vi "Drive Controller.vi"(8 "error in":errorcluster) -> ()   [LabVIEW 2025]
doc: "This VI executes continuously carrying out the current operation and responding to updates or new operation requests. It will often contain the timing or control code that is difficult to place directly in TeleOp. This VI generally opens all sensors and motors and isolates the rest of the robot code from knowing implementation details of how the operations are carried out."
uses:
  <vilib>/Rock Robotics/WPI/Framework/Completion Status.ctl
  Drive Setpoints.ctl
  Drive Operations.ctl
  bordeaux-main/Bordeaux/Types/Single Cmd Info.ctl
  <vilib>/picture/picture.llb/imagedata.ctl
  bordeaux-main/Bordeaux/Types/Trajectory Data.ctl
  bordeaux-main/Bordeaux/Types/Segment Type.ctl
  <vilib>/Rock Robotics/WPI/ThirdParty/REV Robotics/REVLib/Typedef/SPARK PID Gains.ctl
  <vilib>/Rock Robotics/WPI/ThirdParty/REV Robotics/REVLib/Typedef/SPARK Feed Forward Gains.ctl
  <vilib>/Rock Robotics/WPI/ThirdParty/REV Robotics/REVLib/Typedef/Spark MAX Idle Mode.ctl
  <vilib>/Rock Robotics/WPI/ThirdParty/REV Robotics/REVLib/Typedef/Spark MAX Control Type.ctl
  <vilib>/Rock Robotics/WPI/ThirdParty/REV Robotics/REVLib/SubVI/Public/SPARK Open Brushless.vi
  <vilib>/Rock Robotics/WPI/ThirdParty/REV Robotics/REVLib/SubVI/Public/SPARK Configure Power Current Limit.vi
  <vilib>/Rock Robotics/WPI/ThirdParty/REV Robotics/REVLib/SubVI/Public/SPARK Configure Follower Mode From Ref.vi
  <vilib>/Rock Robotics/WPI/ThirdParty/REV Robotics/REVLib/SubVI/Public/SPARK Configure Basic Idle Mode.vi
  <vilib>/Rock Robotics/WPI/ThirdParty/REV Robotics/REVLib/SubVI/Public/SPARK Configure Closed Loop Gains.vi
panel:
  in  "Feed Forward Gains":T1={"kV"=0.00205, "kS"=0.0, "kA"=0.01, "kG"=0.0, "kCos"=0.0, "kCosRatio"=0.0}
  in  "PID Gains":T2={"kP"=1e-05, "kI"=0.0, "kD"=0.0}
  in  "V Scale":dbl=1.0
  in  "Interactive Values":T3
  in  "Buttons":cluster{"Execute Cmd":bool, "Abort Cmd":bool}
  out "Command Timing":cluster{"Start Time (ms)":u32, "Iterations":i32}
  out "Status":T9
  out "Setpoints":T10(graph)
  out "Current\nCmd":string
  # "Interactive Command: You may fill in the settings for a command\nand schedule it with the Execute button. You can observe and abort\nany command while fine tuning the code for the controller."
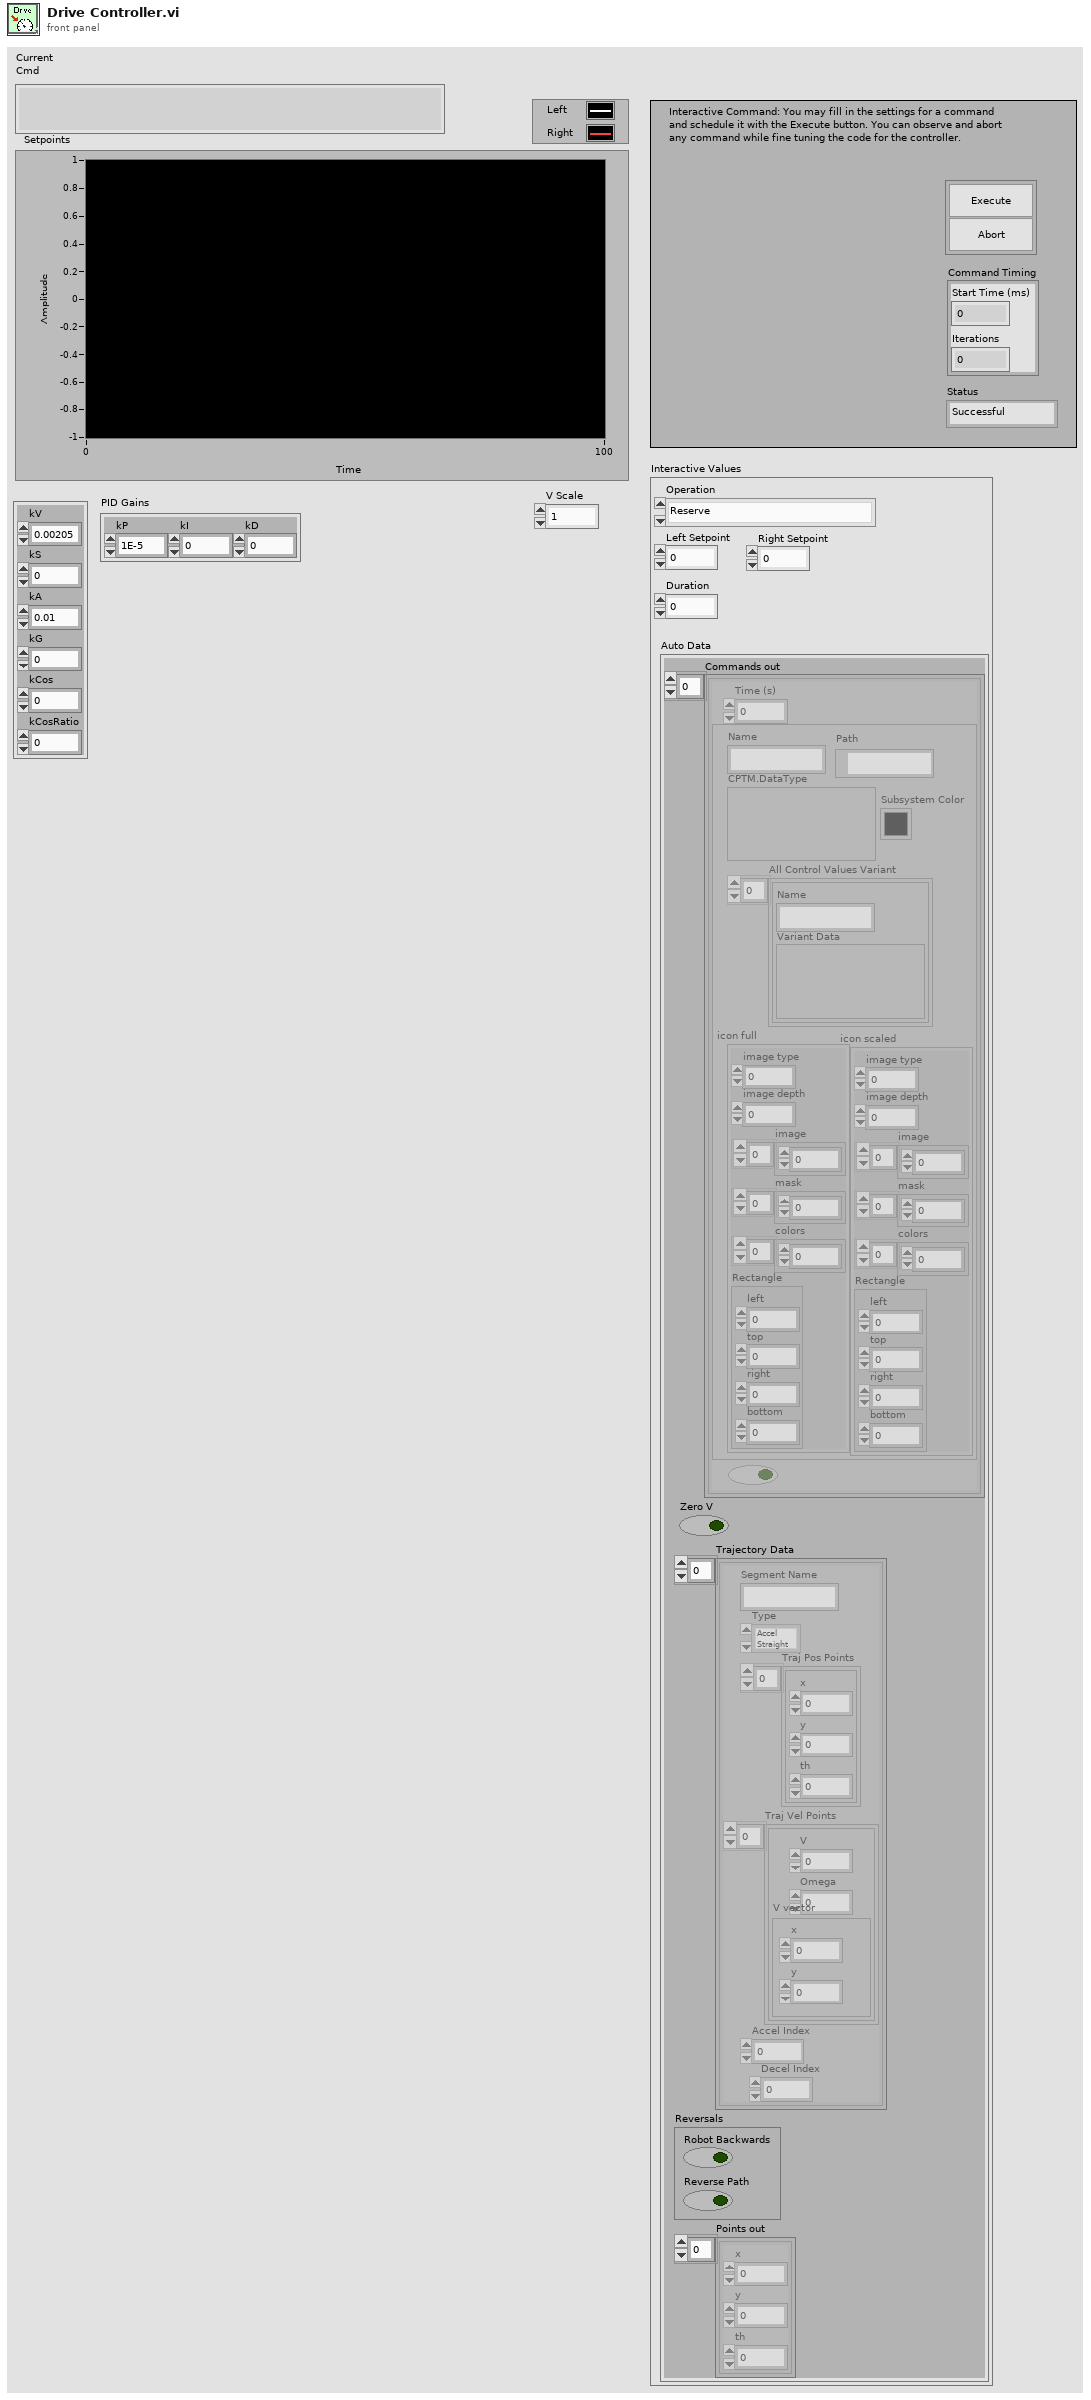
[diagram p1: front panel]
types:
  T1 = typedef "SPARK Feed Forward Gains.ctl" = cluster{"kV":dbl, "kS":dbl, "kA":dbl, "kG":dbl, "kCos":dbl, "kCosRatio":dbl}
  T2 = typedef "SPARK PID Gains.ctl" = cluster{"kP":dbl, "kI":dbl, "kD":dbl}
  T3 = typedef "Drive Setpoints.ctl" = cluster{"Operation":T4, "Left Setpoint":dbl, "Right Setpoint":dbl, "Duration":dbl, "Auto Data":cluster{"Commands out":cluster{"Time (s)":dbl, T5, bool}[], "Zero V":bool, "Trajectory Data":T7, "Reversals":cluster{"Robot Backwards":bool, "Reverse Path":bool}, "Points out":cluster{"x":dbl, "y":dbl, "th":dbl}[]}}
  T4 = typedef "Drive Operations.ctl" = enum16{"Reserve", "Read Current", "Immediate", "Drive for Time", "Play Path", "Drive for Distance", "Turn Aligning"}
  T5 = typedef "Single Cmd Info.ctl" = cluster{"Name":string, "CPTM.DataType":variant, "All Control Values Variant":cluster{"Name":string, "Variant Data":variant}[], "icon full":T6, "icon scaled":T6, "Path":path, "Subsystem Color":u32}
  T6 = typedef "imagedata.ctl" = cluster{"image type":i32, "image depth":i32, "image":u8[], "mask":u8[], "colors":u32[], "Rectangle":cluster{"left":i16, "top":i16, "right":i16, "bottom":i16}}
  T7 = typedef "Trajectory Data.ctl" = cluster{"Segment Name":string, "Type":T8, "Traj Pos Points":cluster{"x":dbl, "y":dbl, "th":dbl}[], "Traj Vel Points":cluster{"V":dbl, "Omega":dbl, "V vector":cluster{"y":dbl, "x":dbl}}[], "Accel Index":i32, "Decel Index":i32}[]
  T8 = typedef "Segment Type.ctl" = enum16{"Accel Straight", "Const Straight", "Blend", "Circle", "Bezier"}
  T9 = typedef "Completion Status.ctl" = enum16{"Successful", "Aborted", "Incomplete"}
  T10 = cluster{"Left Setpoint":dbl, "Right Setpoint":dbl}
  T11 = typedef "Spark MAX Idle Mode.ctl" = enum16{"Coast", "Brake"}
  T12 = typedef "WPI_MotorControlDeviceRef.ctl" = cluster{"DeviceStatus":errorcluster, "Type":T13, "PWM":cluster{"PWM Channel":T14, "DeadBand":T15}, "CAN":cluster{"Device Number":u8, "SetOutput VI Ref":variant, "GetOutput VI Ref":variant, "Enable VI Ref":variant, "Disable VI Ref":variant, "Data":variant}, "Invert":bool, "DIO PWM":cluster{"PWM \"Enable\" Channel":T14, "DIOChannel":T16, "PWM Rate":dbl}}
  T13 = typedef "WPI_MotorControlType.ctl" = enum16{"PWM", "CAN", "DIO PWM"}
  T14 = typedef "FPGA_DIOPWMChannel.ctl" = enum8{"PWM 0", "PWM 1", "PWM 2", "PWM 3", "PWM 4", "PWM 5", "PWM 6", "PWM 7", "PWM 8", "PWM 9", "PWM MXP 0", "PWM MXP 1", "PWM MXP 2", "PWM MXP 3", "PWM MXP 4", "PWM MXP 5", "PWM MXP 6", "PWM MXP 7", "PWM MXP 8", "PWM MXP 9", "Invalid"}
  T15 = typedef "WPI_PWMDeadband.ctl" = cluster{"Name":string, "maxPositivePwm":i32, "minPositivePwm":i32, "centerPwm":i32, "maxNegativePwm":i32, "minNegativePwm":i32, "angularRange":u16}
  T16 = typedef "FPGA_DIOChannel.ctl" = enum8{"DIO 0", "DIO 1", "DIO 2", "DIO 3", "DIO 4", "DIO 5", "DIO 6", "DIO 7", "DIO 8", "DIO 9", "DIO MXP 0", "DIO MXP 1", "DIO MXP 2", "DIO MXP 3", "DIO MXP 4", "DIO MXP 5", "DIO MXP 6", "DIO MXP 7", "DIO MXP 8", "DIO MXP 9", "DIO MXP 10", "DIO MXP 11", "DIO MXP 12", "DIO MXP 13", "DIO MXP 14", "DIO MXP 15", "SPI Port CS1", "SPI Port CS2", "SPI Port CS3", "SPI Port MISO", "SPI Port MOSI", "Invalid"}
  T17 = typedef "Command Status Info.ctl" = cluster{"Name":string, "Status":T9, "notifier out":T18}
  T18 = typedef "Completion Notifier.ctl" = refnum<notifier>
  T19 = cluster{"SubSystem Data":T3, cluster{"Start Time (ms)":u32, "Iterations":i32}, cluster{"Command Info":T17, "Description":string, "Default Command":T3, "queue out":refnum<queue>, "Subsystem Name":string}}
  T20 = cluster{"Commands out":cluster{"Time (s)":dbl, T5, bool}[], "Zero V":bool, "Trajectory Data":T7, "Reversals":cluster{"Robot Backwards":bool, "Reverse Path":bool}, "Points out":cluster{"x":dbl, "y":dbl, "th":dbl}[]}
  T21 = typedef "Spark MAX Control Type.ctl" = enum16{"Percent VBus", "Voltage", "Velocity", "Position", "Smart Motion", "Current", "Smart Velocity", "MAXMotion Position", "MAXMotion Velocity"}
  T22 = cluster{"SubSystem Data":T3, cluster{"Start Time (ms)":u32, "Iterations":i32}, "Default Command Arguments":cluster{"Command Info":T17, "Description":string, "Default Command":T3, "queue out":refnum<queue>, "Subsystem Name":string}}
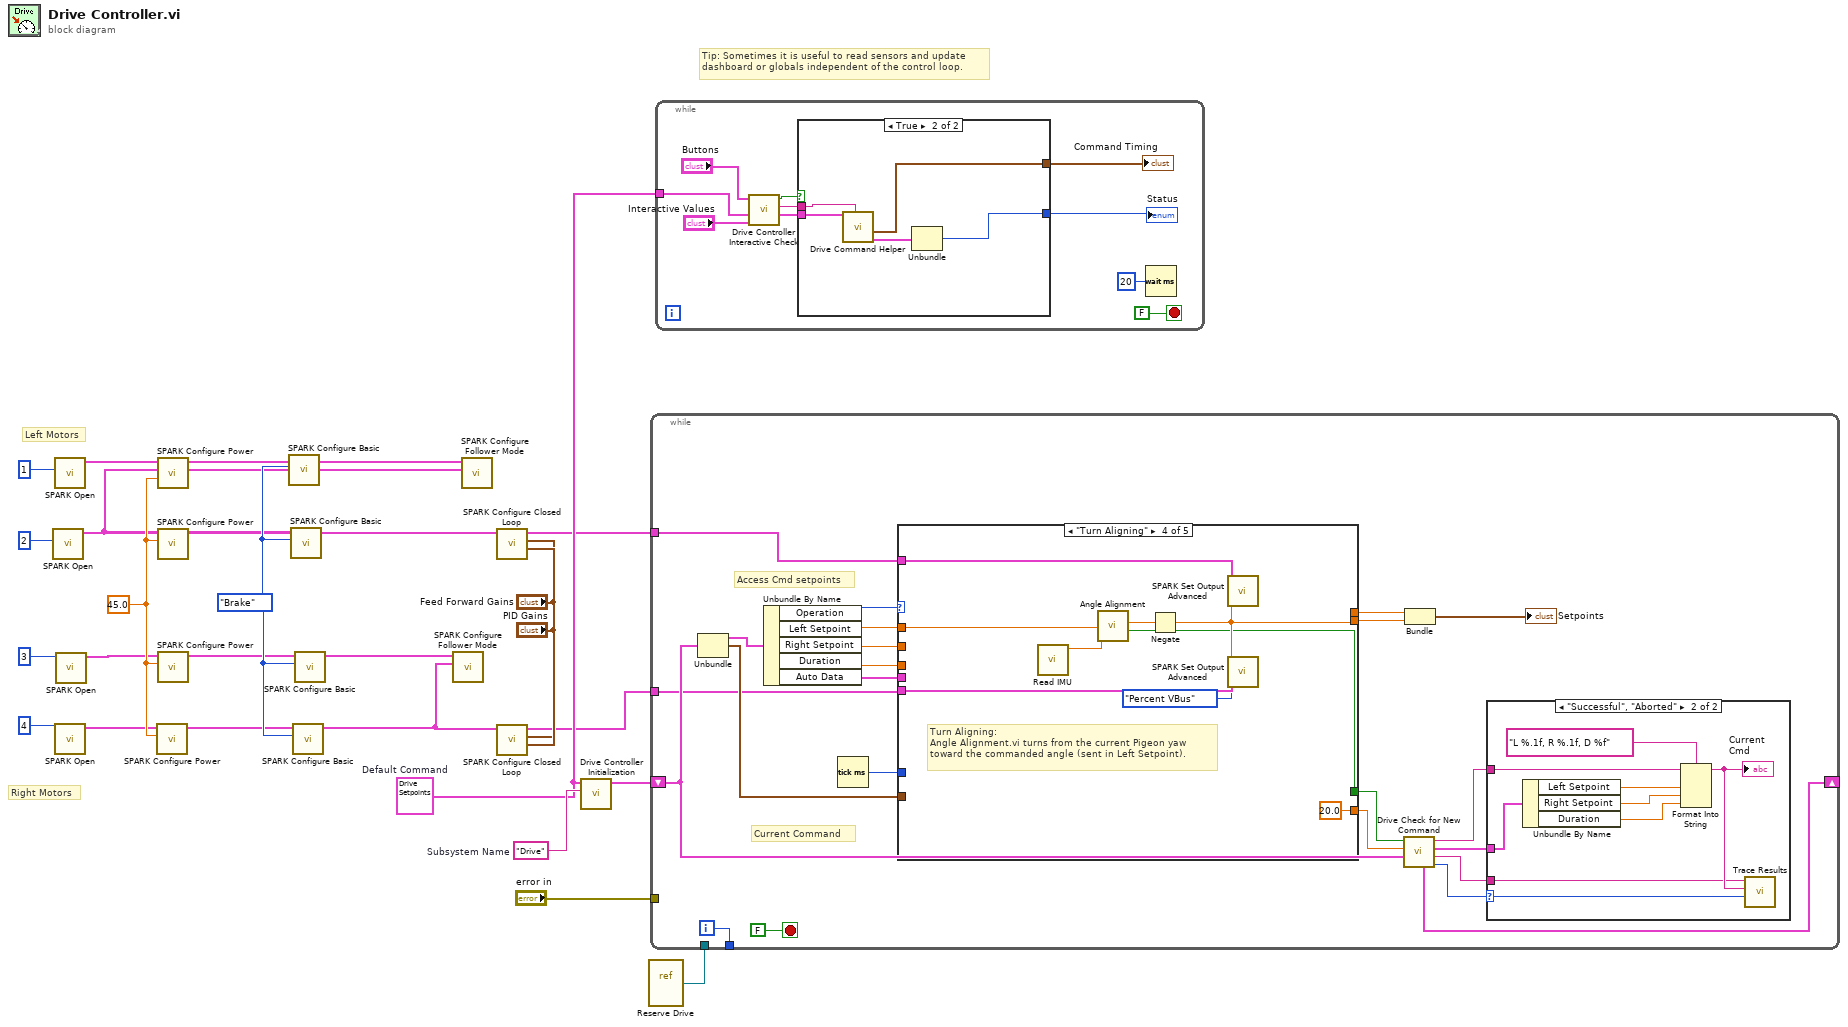
[diagram p0: block diagram]
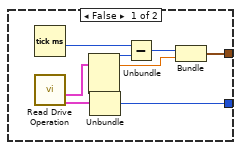
[diagram p2: hidden frame]
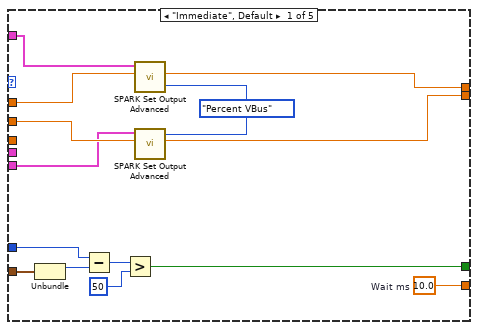
[diagram p4: hidden frame]
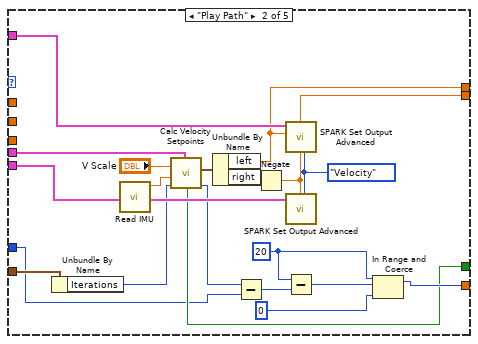
[diagram p5: hidden frame]
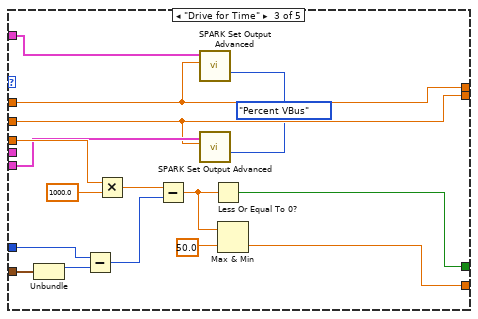
[diagram p6: hidden frame]
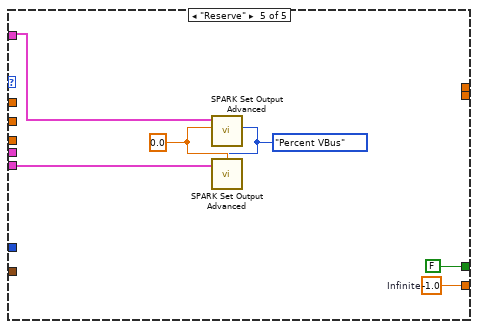
[diagram p7: hidden frame]
diagram:
  w7 = Spark_MAX_Idle_Mode."Brake" ("Idle Mode")
  w8 = 45.0 ("Primay Current Limit (80A)")
  w13 = T3 {"Operation"=enum."Reserve", "Left Setpoint"=0.0, "Right Setpoint"=0.0, "Duration"=0.0, "Auto Data"={"Commands out"=[], "Zero V"=FALSE, "Trajectory Data"=[], "Reversals"={"Robot Backwards"=FALSE, "Reverse Path"=FALSE}, "Points out"=[]}}  # Default Command
  w17 = "Drive"  # Subsystem Name
  # "Right Motors"
  # "Left Motors"
  # "Tip: Sometimes it is useful to read sensors and update\ndashboard or globals independent of the control loop."
  n1 = call-poly <vilib>:"SPARK Open.vi"("Device Number"=u8 2) -> ("MotorControlDeviceRef"=w2:T12)  [unwired: 9 in, 1 out]
  n2 = call-poly <vilib>:"SPARK Open.vi"("Device Number"=u8 1) -> ("MotorControlDeviceRef"=w1:T12)  [unwired: 9 in, 1 out]
  n3 = call-poly <vilib>:"SPARK Open.vi"("Device Number"=u8 4) -> ("MotorControlDeviceRef"=w3:T12)  [unwired: 9 in, 1 out]
  n4 = call-poly <vilib>:"SPARK Open.vi"("Device Number"=u8 3) -> ("MotorControlDeviceRef"=w4:T12)  [unwired: 9 in, 1 out]
  n5 = call-poly <vilib>:"SPARK Configure Power.vi"("Current Limit A (100)"=w8, "MotorControlDeviceRef in"=w3) -> ()  [unwired: 8 in, 2 out]
  n6 = call-poly <vilib>:"SPARK Configure Power.vi"("Current Limit A (100)"=w8, "MotorControlDeviceRef in"=w1) -> ()  [unwired: 8 in, 2 out]
  n7 = call-poly <vilib>:"SPARK Configure Power.vi"("Current Limit A (100)"=w8, "MotorControlDeviceRef in"=w2) -> ()  [unwired: 8 in, 2 out]
  n8 = call-poly <vilib>:"SPARK Configure Power.vi"("Current Limit A (100)"=w8, "MotorControlDeviceRef in"=w4) -> ()  [unwired: 8 in, 2 out]
  n9 = call-poly <vilib>:"SPARK Configure Basic.vi"("Idle Mode"=w7, "MotorControlDeviceRef in"=w1) -> ()  [unwired: 8 in, 2 out]
  n10 = call-poly <vilib>:"SPARK Configure Basic.vi"("Idle Mode"=w7, "MotorControlDeviceRef in"=w2) -> ()  [unwired: 8 in, 2 out]
  n11 = call-poly <vilib>:"SPARK Configure Basic.vi"("Idle Mode"=w7, "MotorControlDeviceRef in"=w3) -> ()  [unwired: 8 in, 2 out]
  n12 = call-poly <vilib>:"SPARK Configure Basic.vi"("Idle Mode"=w7, "MotorControlDeviceRef in"=w4) -> ()  [unwired: 8 in, 2 out]
  n13 = call-poly <vilib>:"SPARK Configure Follower Mode.vi"("Leader MotorControlDeviceRef"=w3, "MotorControlDeviceRef in"=w4) -> ()  [unwired: 8 in, 2 out]
  n14 = call-poly <vilib>:"SPARK Configure Follower Mode.vi"("Leader MotorControlDeviceRef"=w2, "MotorControlDeviceRef in"=w1) -> ()  [unwired: 8 in, 2 out]
  n15 = call-poly <vilib>:"SPARK Configure Closed Loop.vi"("Feed Forward Gains"="Feed Forward Gains", "PID Gains"="PID Gains", "MotorControlDeviceRef in"=w2) -> ()  [unwired: 7 in, 2 out]
  n16 = call-poly <vilib>:"SPARK Configure Closed Loop.vi"("Feed Forward Gains"="Feed Forward Gains", "PID Gains"="PID Gains", "MotorControlDeviceRef in"=w3) -> ()  [unwired: 7 in, 2 out]
  n17 = call "Drive Controller Initialization.vi"("Subsystem Name"=w17, "Default Command"=w13) -> ("Current Command"=w15:T19)  [unwired: 9 in]
  n18 = vi-ref "Reserve Drive.vi"() -> (w14:refnum<vi>)
  n19 = while {
    shift-right: [w28] -> _
    shift-left: w15 -> [w21]
    tunnel: [w39] -> _
    tunnel: "error in" -> [_]
    tunnel: w14 -> [_]
    tunnel: w2 -> [w20]
    tunnel: w3 -> [w19]
    i -> [w39]
    stop <- FALSE stop-if-true
    # "Current Command"
    # "Access Cmd setpoints"
    n20 = Unbundle(w21) -> ("SubSystem Data"=w35:T3, w22:cluster{"Start Time (ms)":u32, "Iterations":i32})  [unwired: 1 out]
    n21 = Unbundle By Name(w35) -> ("Operation"=w34:T4, "Left Setpoint"=w33:dbl, "Right Setpoint"=w32:dbl, "Duration"=w31:dbl, "Auto Data"=w18:T20)
    n22 = Tick Count (ms)() -> (millisecond timer value=w30:u32)
    n23 = case shown="\"Turn Aligning\"" w34 {
      tunnel: [w61 w76 w87 20.0 ("Infinite") w112] -> w27
      tunnel: [w56 w68 w92 w100 FALSE ("ignore previous (F)")] -> w26
      tunnel: w22 -> [w55 w81 w94 _ _]
      tunnel: [w53 w72 w85 w103 _] -> w37
      tunnel: [w52 w70 w83 w103 _] -> w36
      tunnel: w33 -> [w53 _ w85 w105 _]
      tunnel: w32 -> [w52 _ w83 _ _]
      tunnel: w31 -> [_ _ w91 _ _]
      tunnel: w30 -> [w57 w62 w90 _ _]
      tunnel: w20 -> [w54 w75 w86 w102 w110]
      tunnel: w19 -> [w51 w74 w84 w101 w109]
      tunnel: w18 -> [_ w69 _ _ _]
      frame "Immediate", Default {
        w50 = Spark_MAX_Control_Type."Percent VBus" ("Control Mode")
        w61 = 10.0  # Wait ms
        n24 = Unbundle(w55) -> ("Start Time (ms)"=w58:u32)  [unwired: 1 out]
        n25 = Subtract(x=w57, y=w58) -> (x-y=w59:u32)
        n26 = Greater?(x=w59, y=u8 50 ("Left Motor")) -> (0:w56:bool)
        n27 = call <vilib>:"SPARK Set Output Advanced.vi"("Control Mode"=w50, "Setpoint"=w53, "MotorControlDevRef"=w54) -> ()  [unwired: 7 in, 2 out]
        n28 = call <vilib>:"SPARK Set Output Advanced.vi"("Control Mode"=w50, "Setpoint"=w52, "MotorControlDevRef"=w51) -> ()  [unwired: 7 in, 2 out]
      }
      frame "Play Path" {
        w73 = Spark_MAX_Control_Type."Velocity" ("Control Mode")
        w78 = u32 20 ("x")
        n29 = Unbundle By Name(w81) -> ("Iterations"=w66:i32)
        n30 = call "Read IMU.vi"() -> ("Heading"=w64:dbl)  [unwired: 11 in]
        n31 = call "Calc Velocity Setpoints.vi"("Autos"=w69, "Iterations"=w66, "Angle"=w64, "V Scale"="V Scale") -> ("tick count(ms)"=w67:u32, "Finished?"=w68:bool, "setpoints"=w63:cluster{"left":dbl, "right":dbl})  [unwired: 5 in]
        n32 = Unbundle By Name(w63) -> ("left"=w72:dbl, "right"=w71:dbl)
        n33 = Subtract(x=w67, y=w62) -> (x-y=w79:u32)
        n34 = Negate(x=w71) -> (-x=w70:dbl)
        n35 = call <vilib>:"SPARK Set Output Advanced.vi"("Control Mode"=w73, "Setpoint"=w72, "MotorControlDevRef"=w75) -> ()  [unwired: 7 in, 2 out]
        n36 = call <vilib>:"SPARK Set Output Advanced.vi"("Control Mode"=w73, "Setpoint"=w70, "MotorControlDevRef"=w74) -> ()  [unwired: 7 in, 2 out]
        n37 = Subtract(x=w78, y=w79) -> (x-y=w80:u32)
        n38 = In Range and Coerce(upper limit=w78, x=w80, lower limit=u32 0) -> (coerced(x)=w76:u32)  [unwired: 1 out]
      }
      frame "Drive for Time" {
        w82 = Spark_MAX_Control_Type."Percent VBus" ("Control Mode")
        n39 = Unbundle(w94) -> ("Start Time (ms)"=w93:u32)  [unwired: 1 out]
        n40 = Subtract(x=w90, y=w93) -> (x-y=w97:u32)
        n41 = Multiply(x=w91, y=1000.0) -> (x*y=w96:dbl)
        n42 = Subtract(x=w96, y=w97) -> (x-y=w89:dbl)
        n43 = call <vilib>:"SPARK Set Output Advanced.vi"("Control Mode"=w82, "Setpoint"=w85, "MotorControlDevRef"=w86) -> ()  [unwired: 7 in, 2 out]
        n44 = call <vilib>:"SPARK Set Output Advanced.vi"("Control Mode"=w82, "Setpoint"=w83, "MotorControlDevRef"=w84) -> ()  [unwired: 7 in, 2 out]
        n45 = Less Or Equal To 0?(x=w89) -> (x <= 0?=w92:bool)
        n46 = Max & Min(x=w89, y=50.0) -> (min(x,y)=w87:dbl)  [unwired: 1 out]
      }
      frame "Turn Aligning" {
        w99 = Spark_MAX_Control_Type."Percent VBus" ("Control Mode")
        # "Turn Aligning:\nAngle Alignment.vi turns from the current Pigeon yaw\ntoward the commanded angle (sent in Left Setpoint)."
        n47 = call "Read IMU.vi"() -> ("Heading"=w106:dbl)  [unwired: 11 in]
        n48 = call "Angle Alignment.vi"("IMU Reading"=w106, "Setpoint"=w105) -> ("Finished"=w100:bool, "output"=w104:dbl)  [unwired: 8 in]
        n49 = Negate(x=w104) -> (-x=w103:dbl)
        n50 = call <vilib>:"SPARK Set Output Advanced.vi"("Control Mode"=w99, "Setpoint"=w103, "MotorControlDevRef"=w102) -> ()  [unwired: 7 in, 2 out]
        n51 = call <vilib>:"SPARK Set Output Advanced.vi"("Control Mode"=w99, "Setpoint"=w103, "MotorControlDevRef"=w101) -> ()  [unwired: 7 in, 2 out]
      }
      frame "Reserve" {
        w107 = Spark_MAX_Control_Type."Percent VBus" ("Control Mode")
        w108 = 0.0 ("Don't move motors while reserved")
        w112 = -1.0  # Infinite
        n52 = call <vilib>:"SPARK Set Output Advanced.vi"("Control Mode"=w107, "Setpoint"=w108, "MotorControlDevRef"=w110) -> ()  [unwired: 7 in, 2 out]
        n53 = call <vilib>:"SPARK Set Output Advanced.vi"("Control Mode"=w107, "Setpoint"=w108, "MotorControlDevRef"=w109) -> ()  [unwired: 7 in, 2 out]
      }
    }
    n54 = call "Drive Check for New Command.vi"("input cluster"=w21, "Wait time (ms)"=w27, "Finished?"=w26) -> ("Completion"=w29:T9, "Subsystem Name"=w23:string, "Current Command"=w24:T3, "Initial Trace String"=w25:string, "Next Command"=w28:T22)  [unwired: 4 in]
    n55 = Bundle("Left Setpoint"=w37, "Right Setpoint"=w36) -> (→"Setpoints":T10)  [unwired: 1 in]
    n56 = case shown="\"Successful\", \"Aborted\"" w29 {
      selector: w29 -> [_ w49]
      tunnel: w25 -> [_ w44]
      tunnel: w24 -> [_ w45]
      tunnel: w23 -> [_ w41]
      frame "Incomplete", Default {
        # "Continuing current command"
      }
      frame "Successful", "Aborted" {
        # "Report and setup for next command"
        n57 = Unbundle By Name(w45) -> ("Left Setpoint"=w47:dbl, "Right Setpoint"=w48:dbl, "Duration"=w42:dbl)
        n58 = Format Into String(format string="L %.1f, R %.1f, D %f", initial string=w44, w47, w48, w42) -> (resulting string=w43:string)  [unwired: 1 in, 1 out]
        "Current\nCmd" <- w43
        n59 = call <vilib>:"Trace Results.vi"("Status of previous command"=w49, "Description"=w43, "Subsystem"=w41) -> ()  [unwired: 9 in]
      }
    }
  }
  n60 = while {
    tunnel: w13 -> [w114]
    stop <- FALSE stop-if-true
    n61 = call "Drive Controller Interactive Check.vi"("Interactive Command In"="Interactive Values", "Default Command"=w114, "Buttons"="Buttons") -> ("Interactive Command Out"=w116:T3, "Trace String"=w117:string, "Schedule"=w118:bool)  [unwired: 6 in]
    n62 = case shown="True" w118 {
      tunnel: [w127 w135] -> w119
      tunnel: [w126 w131] -> w120
      tunnel: w117 -> [_ w133]
      tunnel: w116 -> [_ w132]
      frame False {
        n63 = Tick Count (ms)() -> (millisecond timer value=w130:u32)
        n64 = call "Read Drive Operation.vi"() -> ("Command Info"=w124:T17, "SubSystem Data"=w123:T3)  [unwired: 9 in, 1 out]
        n65 = Unbundle(w123) -> ("Operation"=w128:T4, "Left Setpoint"=w125:dbl)  [unwired: 3 out]
        n66 = Unbundle(w124) -> ("Status"=w127:T9)  [unwired: 2 out]
        n67 = Subtract(x=w130, y=w128) -> (x-y=w129:u32)
        n68 = Bundle(w129, "Left Setpoint"=w125) -> (w126:cluster{u32, "Left Setpoint":dbl})  [unwired: 1 in]
      }
      frame True {
        n69 = call "Drive Command Helper.vi"("Description"=w133, "SubSystem Data"=w132) -> ("Command Info Out"=w134:T17, "Command Timing"=w131:cluster{"Start Time (ms)":u32, "Iterations":i32})  [unwired: 7 in, 1 out]
        n70 = Unbundle(w134) -> ("Status"=w135:T9)  [unwired: 2 out]
      }
    }
    "Status" <- w119
    "Command Timing" <- w120
    n71 = Wait (ms)(milliseconds to wait=u32 20) -> ()  [unwired: 1 out]
  }
